vi "xnet_canopen_write_od.vi"(8 "error in (no error)":errorcluster, 9 "Value Bytes":u8[](array[numeric]), 10 "OD Index":T1 {"SubIndex" format="%.0x"; "Index" format="%.0x"}, 11 "xnet_co_handle_in":u64) -> (0 "error out":errorcluster, 3 "xnet_co_handle":u64)   [LabVIEW 2023, in "xnet_canopen.lvlib"]
uses:
  typedef/od index.ctl
  <vilib>/Utility/error.llb/Error Cluster From Error Code.vi
  xnet_canopen.lvlib
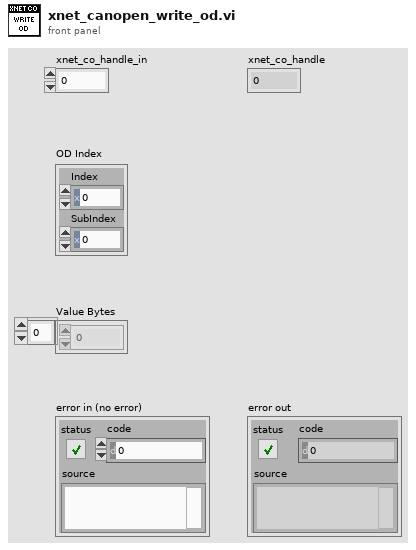
[diagram p1: front panel]
types:
  T1 = typedef "xnet_canopen.lvlib/od index.ctl" = cluster{"Index":u16, "SubIndex":u8}
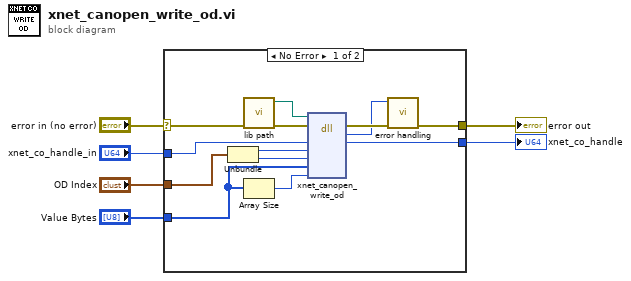
[diagram p0: block diagram]
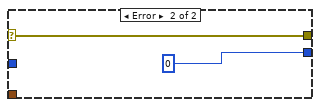
[diagram p2: hidden frame]
diagram:
  n1 = case shown="No Error" "error in (no error)" {
    selector: "error in (no error)" -> [w16 w20]
    tunnel: [w15 w20] -> w5
    tunnel: [w7 u64 0 ("phandle")] -> w4
    tunnel: "xnet_co_handle_in" -> [w17 _]
    tunnel: "OD Index" -> [w14 _]
    tunnel: "Value Bytes" -> [w10 _]
    frame No Error {
      n2 = Unbundle(w14) -> ("Index"=w13:u16, "SubIndex"=w12:u8)
      n3 = call "lib path.vi"() -> ("lib path"=w18:path)  [unwired: 11 in]
      n4 = Array Size(array=w10) -> (size(s)=w9:i32)
      n5 = dll-call lib="?" fn="xnet_canopen_write_od"(path in=w18, error in=w16, "handle"=w17, "index"=w13, "subindex"=w12, "buffer"=w10, "bufsize"=w9) -> (error out=w11:errorcluster, "return type"=w8:i32, "handle"=w7:u64)  [unwired: 5 in, 1 out]
      n6 = call "error handling.vi"("error in (no error)"=w11, "return val"=w8) -> ("error out"=w15:errorcluster)  [unwired: 9 in]
    }
    frame Error {
    }
  }
  "error out" <- w5
  "xnet_co_handle" <- w4
